vi "Test Centric Run Workflow.vi"   [LabVIEW 2020]
uses:
  ed6c40d5-8b85-4fa2-ba7e-ae68b63e62f6.vi
  Nominal Client/Nominal Client.lvclass
  f467e91b-3478-48bd-8c07-4728bc81d03e.vi
  Run/Run.lvclass
  asset/asset.lvclass
  datasources/dataset/dataset.lvclass
  submodules/nominal-streaming-labview-ffi/lv_src/Stream/Stream.lvclass
  submodules/nominal-streaming-labview-ffi/lv_src/Channel/Channel.lvclass
  <vilib>/measure/NI_MABase.lvlib
  99cf41ad-9930-492e-a382-56874d6d0267.vi
  event/event.lvclass
types:
  T1 = enum16{"Sine Wave", "Triangle Wave", "Square Wave", "Sawtooth Wave"}
  T2 = enum16{"Sine Wave", "Triangle Wave", "Square Wave", "Sawtooth Wave"}[]
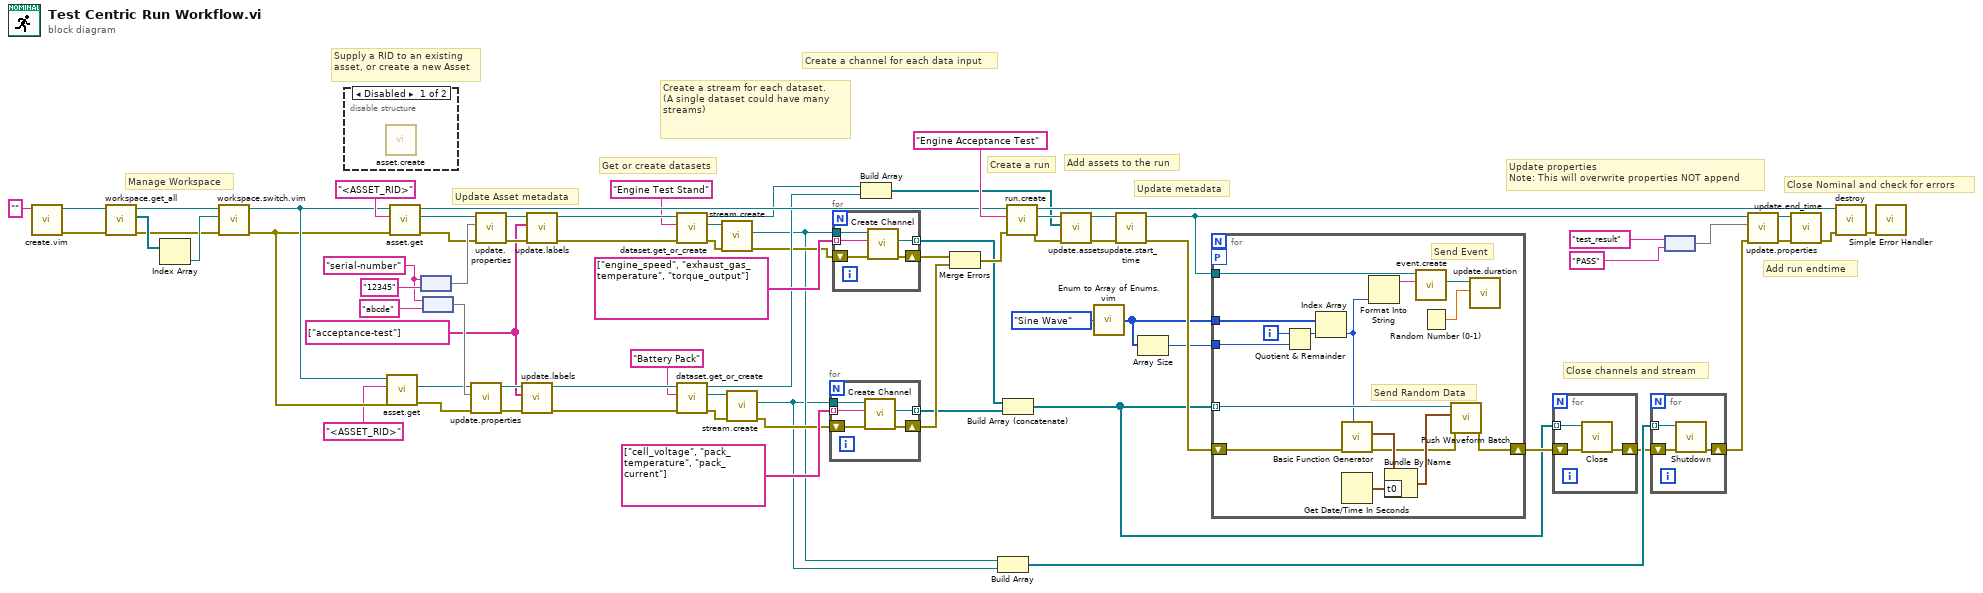
[diagram p0: block diagram]
diagram:
  w55 = string[] ["acceptance-test"] ("labels")
  w72 = "serial-number" ("key")
  # "Close Nominal and check for errors"
  # "Add run endtime"
  # "Update properties\nNote: This will overwrite properties NOT append"
  # "Close channels and stream"
  # "Update metadata"
  # "Add assets to the run"
  # "Create a run"
  # "Create a channel for each data input"
  # "Create a stream for each dataset.\n(A single dataset could have many streams)"
  # "Get or create datasets"
  # "Update Asset metadata"
  # "Supply a RID to an existing asset, or create a new Asset"
  # "Manage Workspace"
  n1 = call "create.vim"("API Token (string or path)"="") -> ("error out"=w64:errorcluster, "Nominal Client"=w66:refnum<class "Nominal Client.lvclass">)  [unwired: 9 in]
  n2 = call "workspace.get_all.vi"("error in"=w64, "Nominal Client in"=w66) -> ("error out"=w65:errorcluster, "Workspaces"=w69:refnum<class "workspace.lvclass">[], "Nominal Client out"=w67:refnum<class "Nominal Client.lvclass">)  [unwired: 7 in]
  n3 = Index Array(array=w69) -> (element=w68:refnum<class "workspace.lvclass">)  [unwired: 1 in]
  n4 = call "workspace.switch.vim"("error in"=w65, "Workspace (Object, RID, Path)"=w68, "Nominal Client in"=w67) -> ("error out"=w43:errorcluster, "Nominal Client out"=w45:refnum<class "Nominal Client.lvclass">)  [unwired: 7 in]
  n5 = disable-structure shown="Disabled" {
    frame Disabled {
      n6 = call "asset.create.vi"() -> ()  [unwired: 9 in, 3 out]
    }
    frame Enabled {
    }
  }
  n7 = call "asset.get.vi"("error in"=w43, "Asset RID"="<ASSET_RID>", "Nominal Client in"=w45) -> ("error out"=w44:errorcluster, "Asset"=w41:refnum<class "asset.lvclass">)  [unwired: 6 in, 1 out]
  n8 = call "asset.get.vi"("error in"=w43, "Asset RID"="<ASSET_RID>", "Nominal Client in"=w45) -> ("error out"=w46:errorcluster, "Asset"=w48:refnum<class "asset.lvclass">, "Nominal Client out"=w47:refnum<class "Nominal Client.lvclass">)  [unwired: 6 in]
  n9 = node(w72, "12345" ("key")) -> (w60:map{string, string})
  n10 = node(w72, "abcde" ("key")) -> (w56:map{string, string})
  n11 = call "update.properties.vi"("error in"=w44, "Properties"=w56, "asset in"=w41) -> ("error out"=w54:errorcluster, "asset out"=w57:refnum<class "asset.lvclass">)  [unwired: 7 in]
  n12 = call "update.properties.vi"("error in"=w46, "Properties"=w60, "asset in"=w48) -> ("error out"=w58:errorcluster, "asset out"=w59:refnum<class "asset.lvclass">)  [unwired: 7 in]
  n13 = call "update.labels.vi"("error in"=w54, "Labels"=w55, "asset in"=w57) -> ("error out"=w51:errorcluster, "asset out"=w50:refnum<class "asset.lvclass">)  [unwired: 7 in]
  n14 = call "update.labels.vi"("error in"=w58, "Labels"=w55, "asset in"=w59) -> ("error out"=w52:errorcluster, "asset out"=w53:refnum<class "asset.lvclass">)  [unwired: 7 in]
  n15 = call "dataset.get_or_create.vi"("error in"=w52, "Datascope Name"="Engine Test Stand" ("Title"), "asset in"=w53) -> ("error out"=w22:errorcluster, "dataset"=w26:refnum<class "dataset.lvclass">, "asset out"=w29:refnum<class "asset.lvclass">)  [unwired: 6 in]
  n16 = call "dataset.get_or_create.vi"("error in"=w51, "Datascope Name"="Battery Pack" ("Title"), "asset in"=w50) -> ("error out"=w21:errorcluster, "dataset"=w25:refnum<class "dataset.lvclass">, "asset out"=w20:refnum<class "asset.lvclass">)  [unwired: 6 in]
  n17 = call "stream.create.vi"("error in (no error)"=w22, "dataset in"=w26) -> ("error out"=w18:errorcluster, "Stream"=w6:refnum<class "Stream.lvclass">)  [unwired: 7 in, 1 out]
  n18 = call "stream.create.vi"("error in (no error)"=w21, "dataset in"=w25) -> ("error out"=w19:errorcluster, "Stream"=w5:refnum<class "Stream.lvclass">)  [unwired: 7 in, 1 out]
  n19 = for {
    tunnel: w5 -> [w78]
    tunnel: string[] ["cell_voltage", "pack_temperature", "pack_current"] -> [w77] mode=indexing
    shift-right: [w75] -> w16
    shift-left: w19 -> [w76]
    tunnel: [w74] -> w12 mode=indexing
    n20 = call "Create Channel.vi"("error in (no error)"=w76, "Channel Name"=w77, "Nominal Streaming in"=w78) -> ("error out"=w75:errorcluster, "Channel"=w74:refnum<class "Channel.lvclass">)  [unwired: 6 in, 1 out]
  }
  n21 = for {
    tunnel: w6 -> [w83]
    tunnel: string[] ["engine_speed", "exhaust_gas_temperature", "torque_output"] -> [w82] mode=indexing
    shift-right: [w81] -> w17
    shift-left: w18 -> [w80]
    tunnel: [w79] -> w13 mode=indexing
    n22 = call "Create Channel.vi"("error in (no error)"=w80, "Channel Name"=w82, "Nominal Streaming in"=w83) -> ("error out"=w81:errorcluster, "Channel"=w79:refnum<class "Channel.lvclass">)  [unwired: 6 in, 1 out]
  }
  n23 = Build Array(w29, w20) -> (w38:refnum<class "asset.lvclass">[])
  n24 = Merge Errors(w17, w16) -> (w15:errorcluster)
  n25 = Build Array(w6, w5) -> (w4:refnum<class "Stream.lvclass">[])
  n26 = Build Array (concatenate)(w13, w12) -> (w7:refnum<class "Channel.lvclass">[])
  n27 = call "run.create.vi"("error in"=w15, "Title"="Engine Acceptance Test" ("Name"), "Nominal Client in"=w47) -> ("error out"=w39:errorcluster, "Run"=w40:refnum<class "Run.lvclass">, "Nominal Client out"=w62:refnum<class "Nominal Client.lvclass">)  [unwired: 6 in]
  n28 = call "update.assets.vi"("error in (no error)"=w39, "Assets"=w38, "Run in"=w40) -> ("error out"=w14:errorcluster, "Run out"=w37:refnum<class "Run.lvclass">)  [unwired: 7 in]
  n29 = call "Enum to Array of Enums.vim"("enum"=T1."Sine Wave" ("signal type")) -> ("array of enums"=w10:T2)
  n30 = call "update.start_time.vi"("error in (no error)"=w14, "Run in"=w37) -> ("error out"=w35:errorcluster, "Run out"=w36:refnum<class "Run.lvclass">)  [unwired: 8 in]
  n31 = Array Size(array=w10) -> (size(s)=w9:i32)
  n32 = for {
    tunnel: w10 -> [w99]
    tunnel: w9 -> [w97]
    shift-right: [w90] -> w8
    shift-left: w35 -> [w93]
    tunnel: w7 -> [w89] mode=indexing
    workers-P: _ -> [_]
    tunnel: w36 -> [w88]
    i -> [w96]
    # "Send Random Data"
    # "Send Event"
    n33 = Quotient & Remainder(x=w96, y=w97) -> (x-y*floor(x/y)=w98:i32)  [unwired: 1 out]
    n34 = Index Array(array=w99, index=w98) -> (element=w87:T1)
    n35 = call <vilib>:"Basic Function Generator.vi"("signal type"=w87, "error in (no error)"=w93) -> ("error out"=w91:errorcluster, "signal out"=w95:waveform(dbl))  [unwired: 7 in, 1 out]
    n36 = Get Date/Time In Seconds() -> (seconds since 1Jan1904=w94:timestamp)
    n37 = Format Into String(w87) -> (resulting string=w86:string)  [unwired: 3 in, 1 out]
    n38 = Bundle By Name(cluster=w95, "t0"=w94) -> (w92:waveform(dbl))
    n39 = call "event.create.vi"("Name"=w86, "Run in"=w88) -> ("event"=w85:refnum<class "event.lvclass">)  [unwired: 7 in, 2 out]
    n40 = Random Number (0-1)() -> (number: 0 to 1=w84:dbl)
    n41 = call "Push Waveform Batch.vi"("error in (no error)"=w91, "Waveform"=w92, "Channel in"=w89) -> ("error out"=w90:errorcluster)  [unwired: 7 in, 1 out]
    n42 = call "update.duration.vi"("Duration (s)"=w84, "event in"=w85) -> ()  [unwired: 8 in, 2 out]
  }
  n43 = for {
    tunnel: w7 -> [w101] mode=indexing
    shift-right: [w100] -> w3
    shift-left: w8 -> [w102]
    n44 = call "Close.vi"("error in (no error)"=w102, "Channel in"=w101) -> ("error out"=w100:errorcluster)  [unwired: 9 in]
  }
  n45 = for {
    shift-right: [w103] -> w2
    shift-left: w3 -> [w105]
    tunnel: w4 -> [w104] mode=indexing
    n46 = call "Shutdown.vi"("error in (no error)"=w105, "Nominal Streaming in"=w104) -> ("error out"=w103:errorcluster)  [unwired: 8 in, 1 out]
  }
  n47 = node("test_result" ("key"), "PASS" ("key")) -> (w30:map{string, string})
  n48 = call "update.properties.vi"("error in (no error)"=w2, "properties"=w30, "Run in"=w36) -> ("error out"=w33:errorcluster, "Run out"=w34:refnum<class "Run.lvclass">)  [unwired: 7 in]
  n49 = call "update.end_time.vi"("error in (no error)"=w33, "Run in"=w34) -> ("error out"=w63:errorcluster)  [unwired: 8 in, 1 out]
  n50 = call "destroy.vi"("error in"=w63, "Nominal Client"=w62) -> ("error out"=w1:errorcluster)  [unwired: 9 in]
  n51 = call <vilib>:"Simple Error Handler.vi"("error in (no error)"=w1) -> ()  [unwired: 4 in, 5 out]
